vi "RealTime.vi"() -> ()   [LabVIEW 2019]
uses:
  ByteGSAPIBase/LimsTestStep/acquisitions.ctl
  <vilib>/Bytelabs/ByteChannelsSetting/ChannelSettingsLib/ChannelsRepos/ChannelsRepoXML/ChannelsRepoXML.lvclass
  C:/Program Files (x86)/National Instruments/LabVIEW 2019/vi.lib/Bytelabs/ByteChannelsSetting/ChannelSettingsLib/ChannelsRepos/ChannelsRepoBase/ChannelsRepoBase.lvclass
  TypeDef/ChannelInfo.ctl
  ByteGSAPIBase/ByteGSAPIBase.lvclass
  TypeDef/TCPMessage.ctl
  <vilib>/Bytelabs/ByteChannelsSetting/ChannelSettingsLib/ChannelsClasses/ChannelBase/ChannelBase.lvclass/ChannelBase.ctl
  <vilib>/Bytelabs/ByteChannelsSetting/ChannelSettingsLib/ChannelsClasses/ChannelAnalog/AnalogRio/AnalogRio.lvclass
  C:/Program Files (x86)/National Instruments/LabVIEW 2019/vi.lib/Bytelabs/ByteChannelsSetting/ChannelSettingsLib/ChannelsClasses/ChannelAnalog/AnalogIn/AnalogIn.lvclass
  ByteGSAPIBase/UpdateChannelsList/fields.ctl
  ByteGSAPIBase/TypeDef/StepAcquisition.ctl
  ByteGSAPIBase/TypeDef/Asset.ctl
  <vilib>/Bytelabs/ByteTCP/TCP_Class/TCP.lvclass
  <vilib>/Bytelabs/ByteSimpleQ/ByteSimpleQ/ByteSimpleQ.lvlib
  <vilib>/Bytelabs/ByteChannelsSetting/ChannelSettingsLib/ChannelsRepos/ChannelsRepoBase/ChannelsRepoBase.lvclass
  <vilib>/Bytelabs/ByteChannelsSetting/ChannelSettingsLib/ChannelsClasses/ChannelBase/ChannelBase.lvclass
panel:
  out "error out":errorcluster
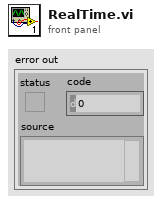
[diagram p1: front panel]
types:
  T1 = typedef "ChannelInfo.ctl" = cluster{"Tag":string, "HW Resource":string, "Raw":dbl}
  T2 = typedef "ByteGSWebAPI.lvlib/ByteGSAPIBase.lvclass/acquisitions.ctl" = cluster{"tags":cluster{"step_id":i32, "test_slug":string, "asset_slug":string}, "acquisitions":cluster{"timestamp":string, "fields":cluster{"name":string, "value":dbl}[]}[]}
  T3 = cluster{"queue out":refnum<queue>, "Acquisitions":T2, "Info":T1[], "TCP_Class":refnum<class "TCP.lvclass">, "Continous?":bool, "Duration":dbl, "ByteGSAPIBase in":refnum<class "ByteGSAPIBase.lvclass">}
  T4 = cluster{"Acquisitions":T2, "Info":T1[], "ByteGSAPIBase in":refnum<class "ByteGSAPIBase.lvclass">, "TCP_Class":refnum<class "TCP.lvclass">}
  T5 = cluster{"ByteGSAPIBase in":refnum<class "ByteGSAPIBase.lvclass">, "TCP_Class":refnum<class "TCP.lvclass">, "ChannelsRepoBase out":refnum<class "ChannelsRepoXML.lvclass">, "queue out":refnum<queue>, "Slug":string, "queue out":refnum<queue>}
  T6 = cluster{"ChannelsRepoBase out":refnum<class "ChannelsRepoXML.lvclass">, "channels":string[], "Duration":dbl, "id":i32, "prova.slug":string, "Continous?":bool, "ByteGSAPIBase in":refnum<class "ByteGSAPIBase.lvclass">}
  T7 = cluster{"timestamp":string, "fields":cluster{"name":string, "value":dbl}[]}
  T8 = typedef "TCPMessage.ctl" = cluster{"Message":string, "Data":variant}
  T9 = cluster{"timestamp":string, "fields":cluster{"name":string, "value":dbl}[]}[]
  T10 = cluster{"ChannelsRepoBase out":refnum<class "ChannelsRepoXML.lvclass">, "channels":string[], "asset_slug":string, "ByteGSAPIBase in":refnum<class "ByteGSAPIBase.lvclass">}
  T11 = typedef "ByteGSWebAPI.lvlib/ByteGSAPIBase.lvclass/fields.ctl" = cluster{"asset_slug":string, "fields":string[]}
  T12 = typedef "ByteGSWebAPI.lvlib/ByteGSAPIBase.lvclass/StepAcquisition.ctl" = cluster{"id":i32, "descrizione":string, "prova":cluster{"slug":string}, "assets":T13[], "criterio_accettazione":string, "valore_criterio_accettazione_max":dbl, "valore_criterio_accettazione_min":dbl, "udm_criterio_accettazione":string, "duration_prova":string, "udm_duration_prova":string, "valore_prova":dbl, "ordine":i32, "user":i32, "link_automation":string, "instruction_automation":string, "data_completamento_checklist":timestamp, "outcome":bool, "step_type":string, "channels":string[]}
  T13 = typedef "ByteGSWebAPI.lvlib/ByteGSAPIBase.lvclass/Asset.ctl" = cluster{"descrizione":string, "slug":string, "id":i32}
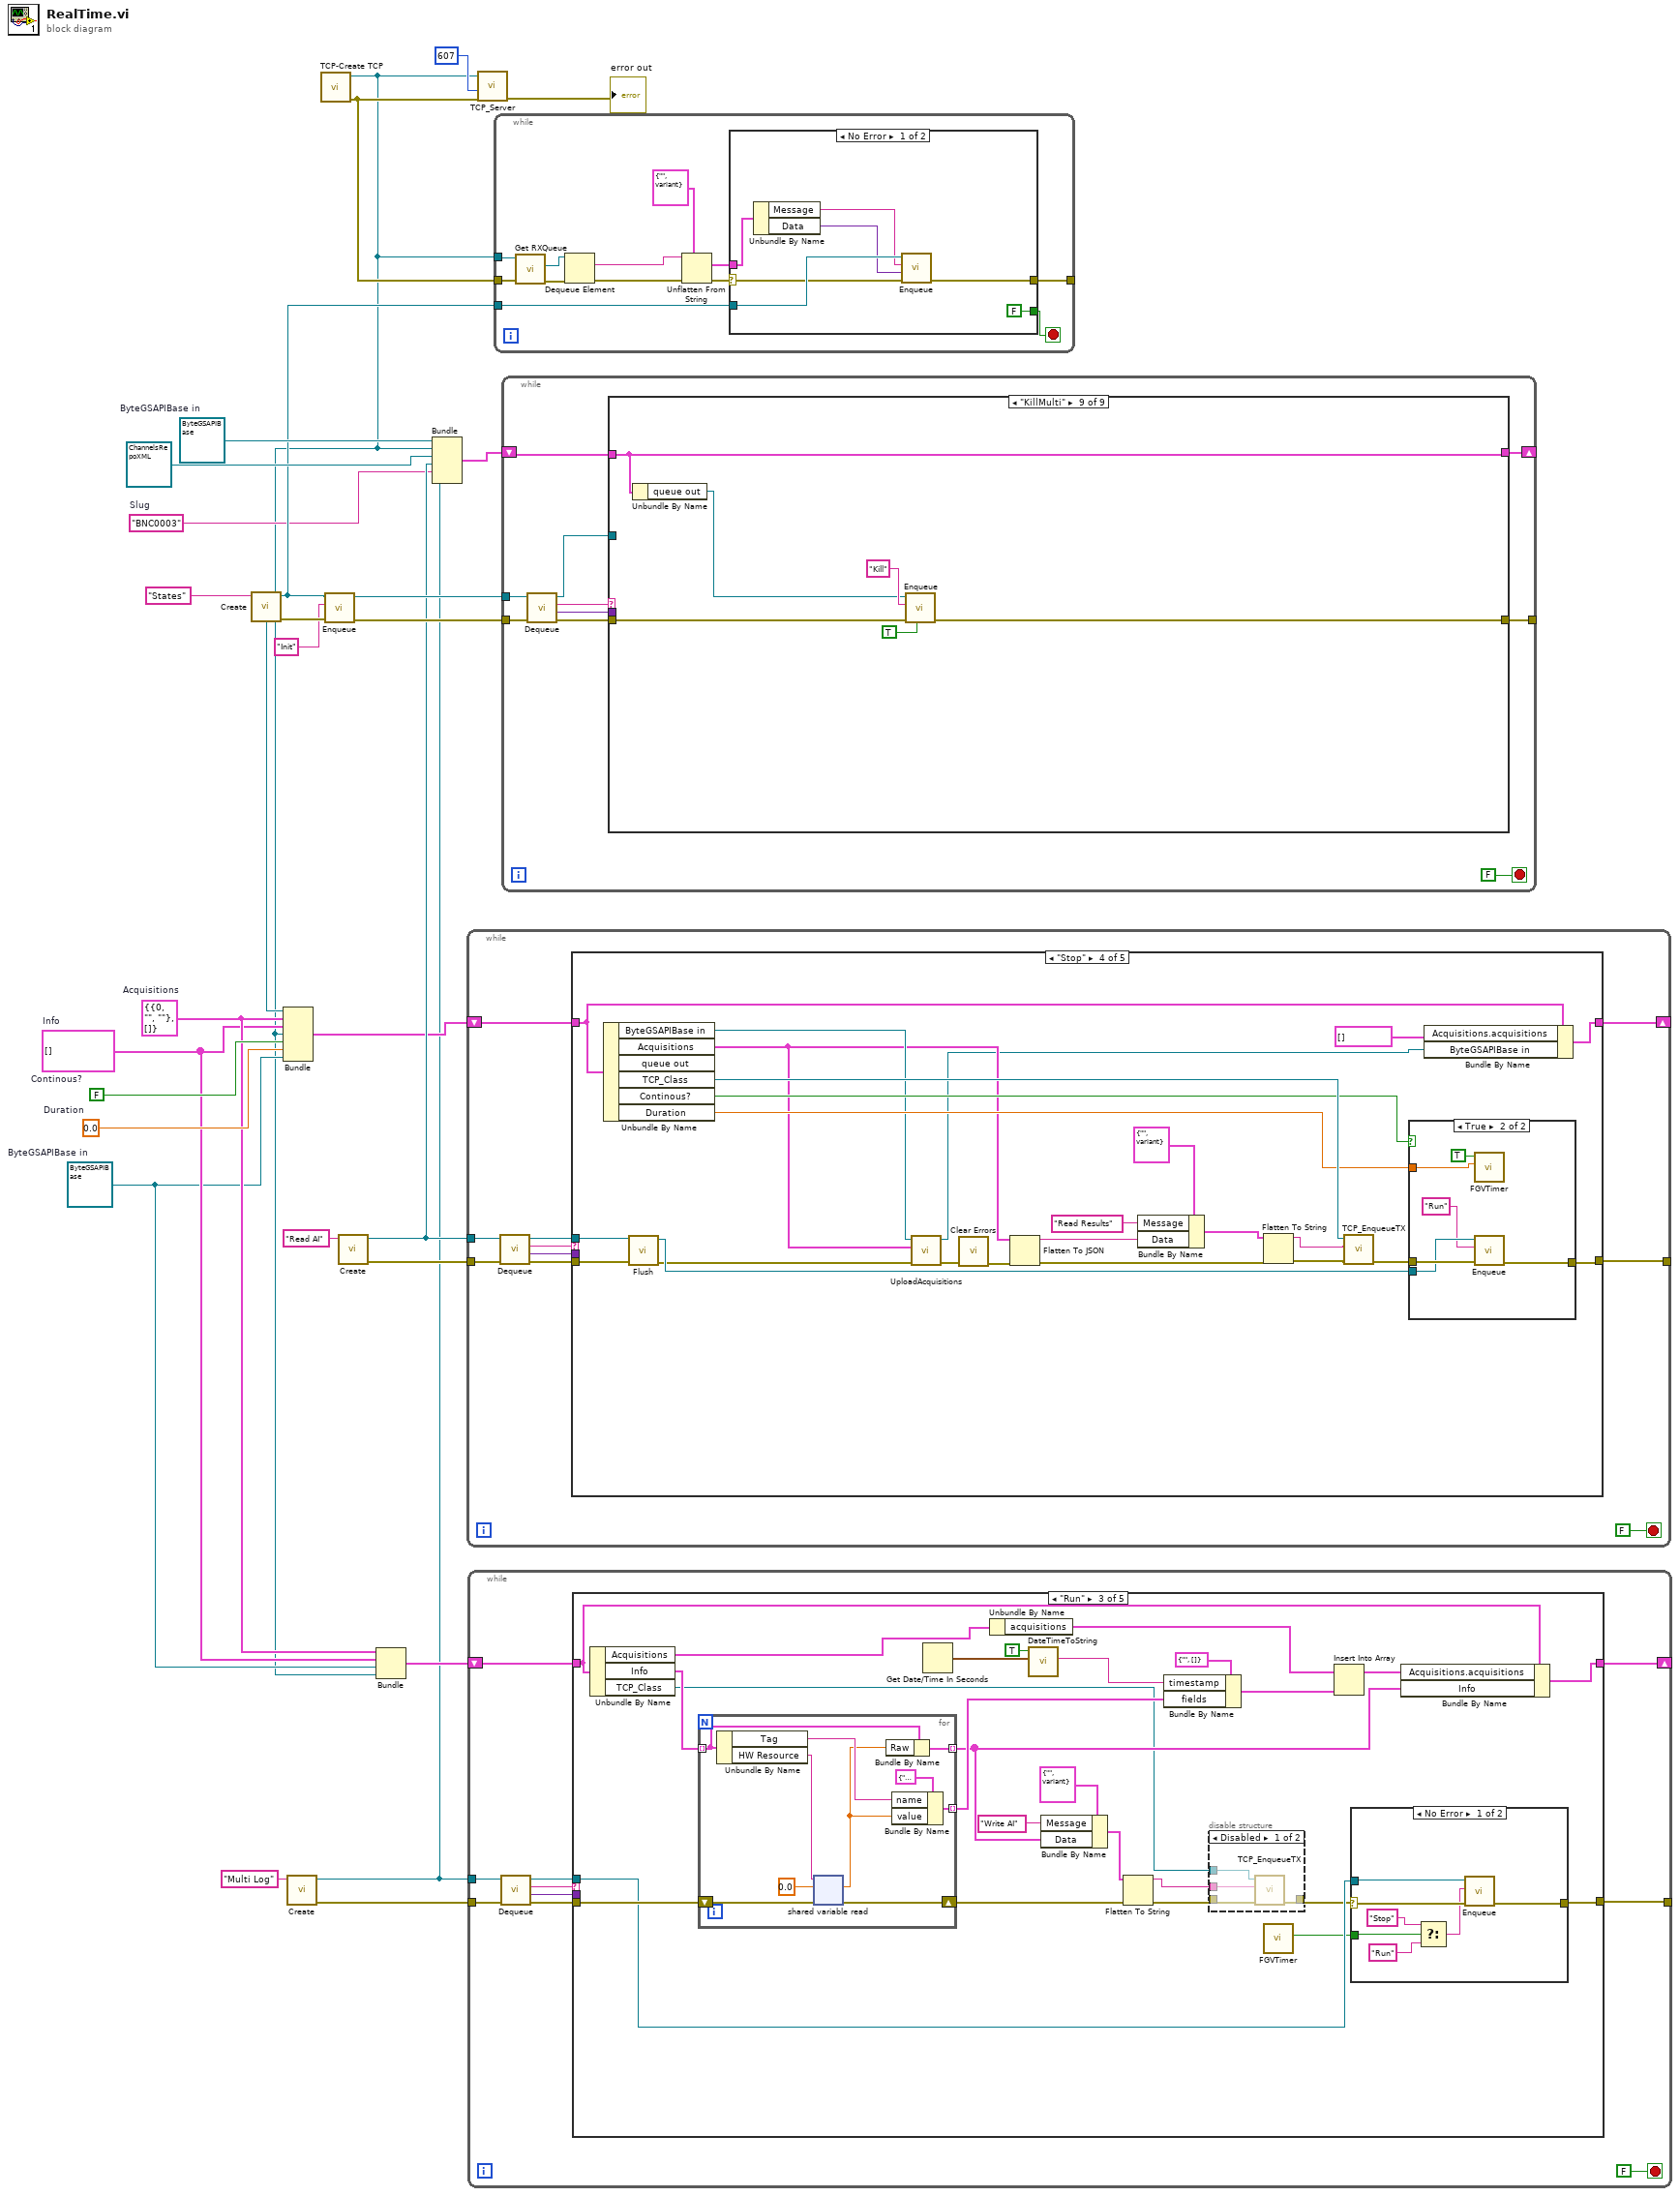
[diagram p0: block diagram]
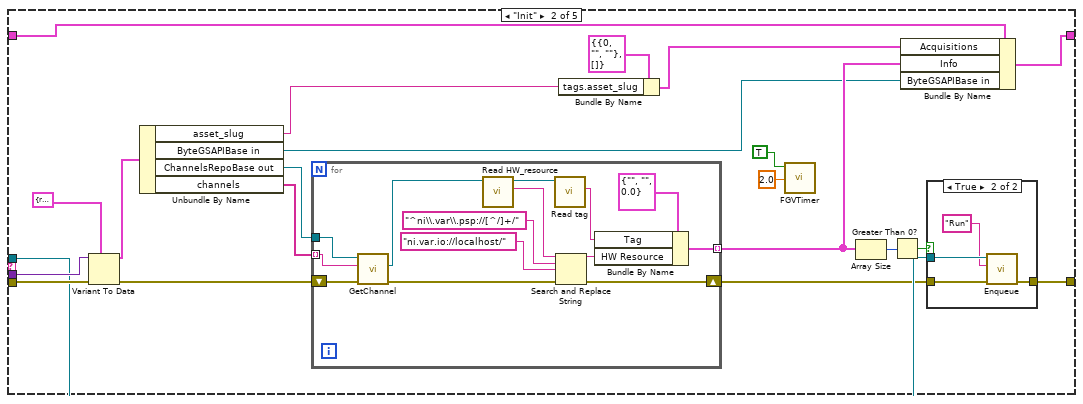
[diagram p3: hidden frame]
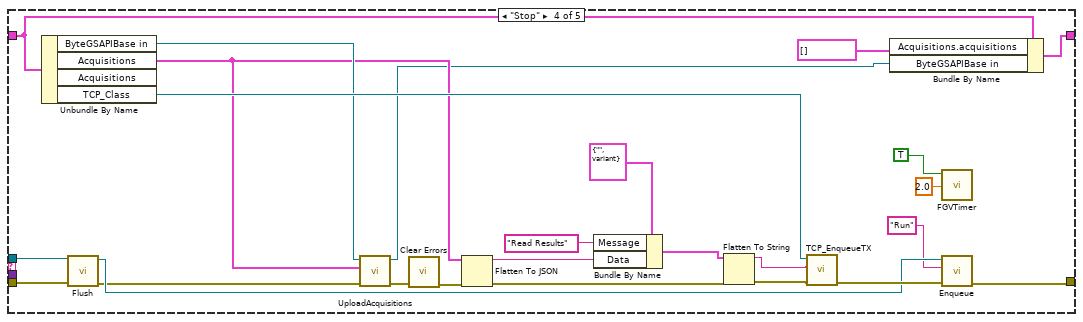
[diagram p7: hidden frame]
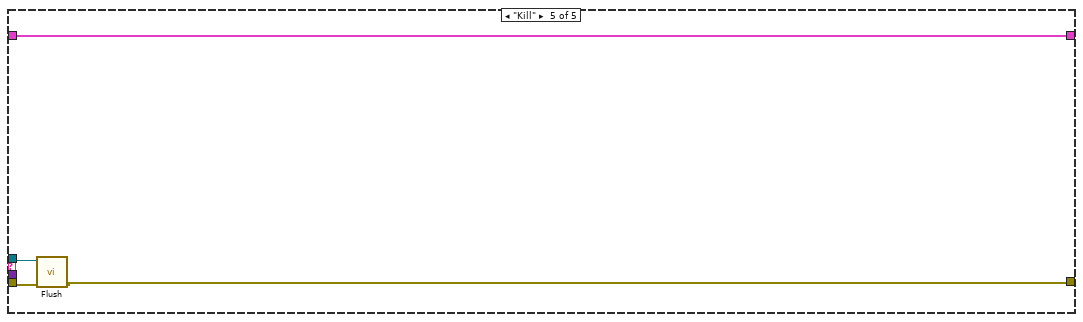
[diagram p8: hidden frame]
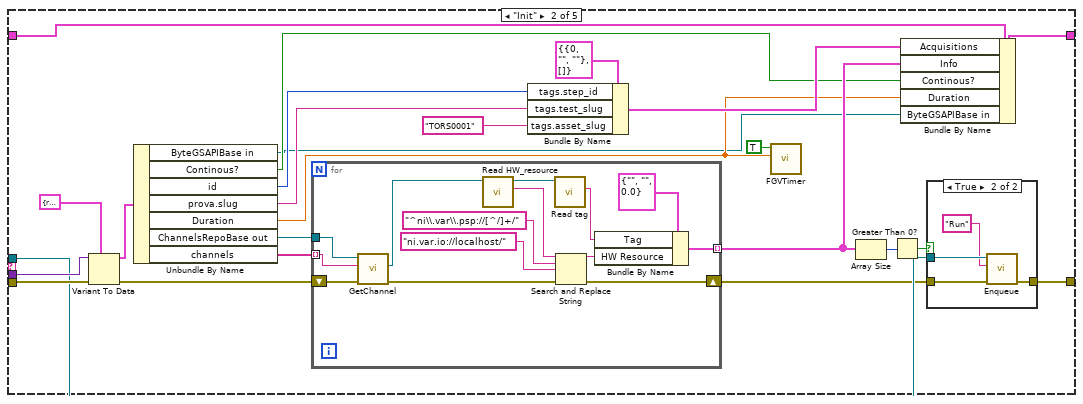
[diagram p10: hidden frame]
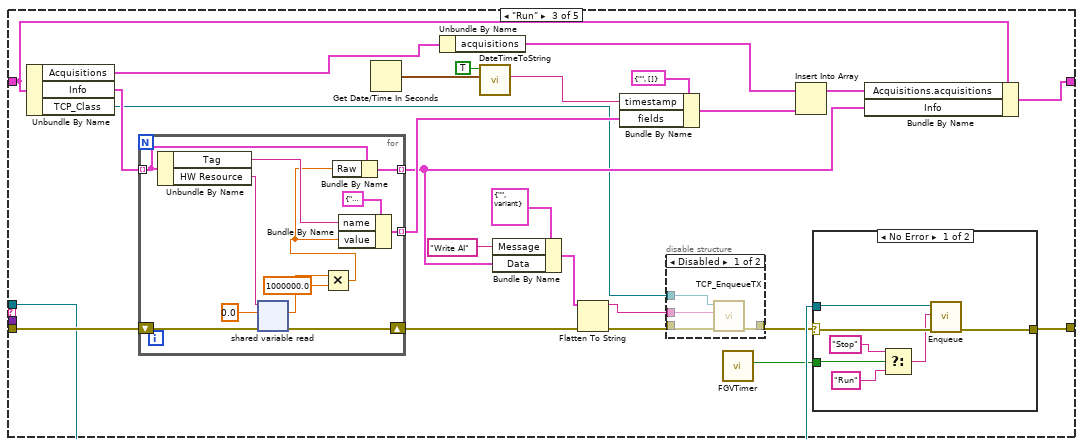
[diagram p12: hidden frame]
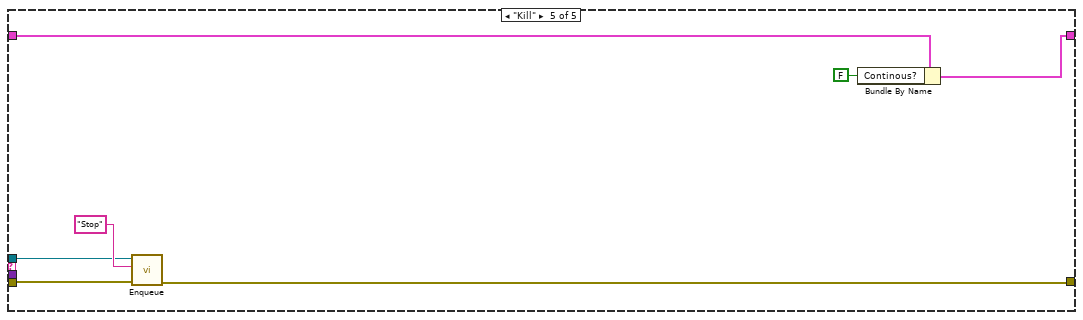
[diagram p16: hidden frame]
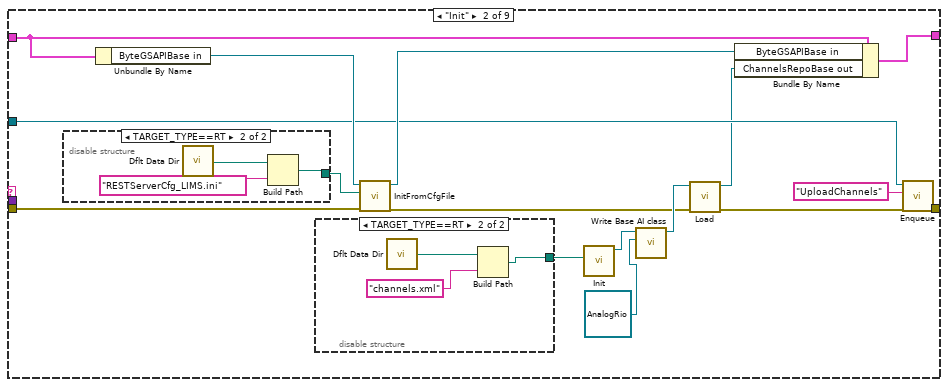
[diagram p18: hidden frame]
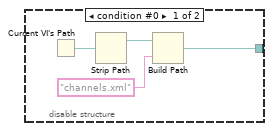
[diagram p19: hidden frame]
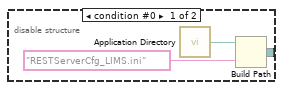
[diagram p20: hidden frame]
diagram:
  w9 = "BNC0003"  # Slug
  w4 = refnum<class "ByteGSAPIBase.lvclass"> refnum  # ByteGSAPIBase in
  w10 = 0.0  # Duration
  w11 = FALSE  # Continous?
  w5 = T1[] []  # Info
  w6 = T2 {"tags"={"step_id"=0, "test_slug"="", "asset_slug"=""}, "acquisitions"=[]}  # Acquisitions
  w17 = refnum<class "ByteGSAPIBase.lvclass"> refnum  # ByteGSAPIBase in
  n1 = call <vilib>:"Create.vi"("name (unnamed)"="States") -> ("error out"=w21:errorcluster, "queue out"=w13:refnum<queue>)  [unwired: 8 in, 1 out]
  n2 = call <vilib>:"Create.vi"("name (unnamed)"="Multi Log") -> ("error out"=w7:errorcluster, "queue out"=w1:refnum<queue>)  [unwired: 8 in, 1 out]
  n3 = call <vilib>:"TCP-Create TCP.vi"() -> ("error out"=w27:errorcluster, "TCP_Class"=w3:refnum<class "TCP.lvclass">)  [unwired: 9 in, 1 out]
  n4 = Bundle("queue out"=w13, "Acquisitions"=w6, "Info"=w5, "TCP_Class"=w3, "Continous?"=w11, "Duration"=w10, "ByteGSAPIBase in"=w4) -> (w12:T3)  [unwired: 1 in]
  n5 = call <vilib>:"Enqueue.vi"("error in (no error)"=w21, "message"="Init", "queue in"=w13) -> ("error out"=w20:errorcluster, "queue out"=w19:refnum<queue>)  [unwired: 6 in, 1 out]
  n6 = call <vilib>:"Create.vi"("name (unnamed)"="Read AI") -> ("error out"=w23:errorcluster, "queue out"=w15:refnum<queue>)  [unwired: 8 in, 1 out]
  n7 = Bundle("Acquisitions"=w6, "Info"=w5, "ByteGSAPIBase in"=w4, "TCP_Class"=w3) -> (w2:T4)  [unwired: 1 in]
  n8 = Bundle("ByteGSAPIBase in"=w17, "TCP_Class"=w3, "ChannelsRepoBase out"=refnum<class "ChannelsRepoXML.lvclass"> refnum, "queue out"=w15, "Slug"=w9, "queue out"=w1) -> (w14:T5)  [unwired: 1 in]
  n9 = while {
    tunnel: w15 -> [w37]
    shift-right: [w28] -> _
    shift-left: w12 -> [w29]
    tunnel: w23 -> [w36]
    tunnel: [w31] -> _
    stop <- FALSE stop-if-true
    n10 = call <vilib>:"Dequeue.vi"("error in (no error)"=w36, "queue in"=w37) -> ("error out"=w35:errorcluster, "data"=w33:variant, "message"=w34:string, "queue out"=w32:refnum<queue>)  [unwired: 5 in, 1 out]
    n11 = case shown="\"Stop\"" w34 {
      tunnel: w35 -> [w39 w63 w107 w155 w168]
      tunnel: w33 -> [_ w62 _ _ _]
      tunnel: w32 -> [_ w58 w106 w154 w167]
      tunnel: [w39 w57 w105 w143 w166] -> w31
      tunnel: w29 -> [w38 w48 w86 w140 w165]
      tunnel: [w38 w46 w84 w139 w163] -> w28
      frame Default {
      }
      frame "Init" {
        n12 = Variant To Data(error in=w63, type=T6 {"ChannelsRepoBase out"=refnum, "channels"=[], "Duration"=0.0, "id"=0, "prova.slug"="", "Continous?"=FALSE, "ByteGSAPIBase in"=refnum} ("output cluster"), Variant=w62) -> (data=w56:T6, error out=w61:errorcluster)
        n13 = Unbundle By Name(w56) -> ("ByteGSAPIBase in"=w40:refnum<class "ByteGSAPIBase.lvclass">, "Continous?"=w44:bool, "id"=w50:i32, "prova.slug"=w49:string, "Duration"=w42:dbl, "ChannelsRepoBase out"=w54:refnum<class "ChannelsRepoXML.lvclass">, "channels"=w55:string[])
        n14 = for {
          shift-right: [w77] -> w53
          shift-left: w61 -> [w72]
          tunnel: [w74] -> w45 mode=indexing
          tunnel: w55 -> [w70] mode=indexing
          tunnel: w54 -> [w73]
          n15 = call <vilib>:"GetChannel.vi"("error in (no error)"=w72, "tag"=w70, "ChannelsRepoBase in"=w73) -> ("error out"=w71:errorcluster, "channel"=w69:refnum<class "ChannelBase.lvclass">)  [unwired: 5 in, 2 out]
          n16 = call <vilib>:"Read HW_resource.vi"("ChannelBase in"=w69) -> ("HW_resource"=w82:string, "ChannelBase out"=w79:refnum<class "ChannelBase.lvclass">)  [unwired: 9 in]
          n17 = call <vilib>:"Read tag.vi"("ChannelBase in"=w79) -> ("tag"=w78:string)  [unwired: 9 in, 1 out]
          n18 = Search and Replace String(input string=w82, search string="^ni\\.var\\.psp://[^/]+/", replace string="ni.var.io://localhost/" ("replace string (\"\")"), error in=w71) -> (result string=w76:string, error out=w77:errorcluster)  [unwired: 4 in, 2 out]
          n19 = Bundle By Name(cluster=T1 {"Tag"="", "HW Resource"="", "Raw"=0.0} ("output cluster"), "Tag"=w78, "HW Resource"=w76) -> (w74:T1)
        }
        n20 = Bundle By Name(cluster=T2 {"tags"={"step_id"=0, "test_slug"="", "asset_slug"=""}, "acquisitions"=[]} ("Cluster"), "tags.step_id"=w50, "tags.test_slug"=w49, "tags.asset_slug"="TORS0001") -> (w47:T2)
        n21 = call "FGVTimer.vi"("set timer"=w42, "Reset"=TRUE) -> ()  [unwired: 8 in, 2 out]
        n22 = Array Size(array=w45) -> (size(s)=w60:i32)
        n23 = Greater Than 0?(x=w60) -> (x > 0?=w59:bool)
        n24 = Bundle By Name(cluster=w48, "Acquisitions"=w47, "Info"=w45, "Continous?"=w44, "Duration"=w42, "ByteGSAPIBase in"=w40) -> (w46:T3)
        n25 = case shown="True" w59 {
          tunnel: w58 -> [_ w68]
          tunnel: [w64 w66] -> w57
          tunnel: w53 -> [w64 w65]
          frame False {
          }
          frame True {
            n26 = call <vilib>:"Enqueue.vi"("error in (no error)"=w65, "message"="Run", "queue in"=w68) -> ("error out"=w66:errorcluster)  [unwired: 6 in, 2 out]
          }
        }
      }
      frame "Run" {
        n27 = Unbundle By Name(w86) -> ("Acquisitions"=w87:T2, "Info"=w88:T1[], "TCP_Class"=w83:refnum<class "TCP.lvclass">)
        n28 = for {
          shift-right: [w127] -> w94
          shift-left: w107 -> [w131]
          tunnel: w88 -> [w128] mode=indexing
          tunnel: [w126] -> w85 mode=indexing
          tunnel: [w123] -> w100 mode=indexing
          n29 = Unbundle By Name(w128) -> ("Tag"=w124:string, "HW Resource"=w129:string)
          n30 = shared-variable-read(w129, w131, 0.0) -> (w127:errorcluster, w122:dbl)  [unwired: 2 out]
          n31 = Multiply(x=w122, y=1000000.0) -> (x*y=w120:dbl)
          n32 = Bundle By Name(cluster=w128, "Raw"=w120) -> (w126:T1)
          n33 = Bundle By Name(cluster=cluster{"name":string, "value":dbl} {"name"="", "value"=0.0} ("fields"), "name"=w124, "value"=w120) -> (w123:cluster{"name":string, "value":dbl})
        }
        n34 = Get Date/Time In Seconds() -> (seconds since 1Jan1904=w91:timestamp)
        n35 = Unbundle By Name(w87) -> ("acquisitions"=w98:T9)
        n36 = call "DateTimeToString.vi"("current time"=w91, "include Time?"=TRUE) -> ("date string"=w90:string)  [unwired: 8 in, 1 out]
        n37 = Bundle By Name(cluster=T8 {"Message"="", "Data"=variant}, "Message"="Write AI", "Data"=w85) -> (w103:T8)
        n38 = Flatten To String(anything=w103, error in (no error)=w94) -> (data string=w95:string, error out=w96:errorcluster)  [unwired: 2 in, 1 out]
        n39 = Bundle By Name(cluster=T7 {"timestamp"="", "fields"=[]} ("acquisition"), "timestamp"=w90, "fields"=w100) -> (w99:T7)
        n40 = disable-structure shown="Disabled" {
          disable-tunnel: w96 -> [w111 _]
          disable-tunnel: w95 -> [w110 _]
          disable-tunnel: [w109 _] -> w92
          disable-tunnel: w83 -> [w108 _]
          frame Disabled {
            n41 = call-dynamic "TCP_EnqueueTX.vi"("error in (no error)"=w111, "Msg to Transmit"=w110, "TCP in"=w108) -> ("error out"=w109:errorcluster)  [unwired: 7 in, 1 out]
          }
          frame Enabled {
          }
        }
        n42 = call "FGVTimer.vi"() -> ("Elapsed?"=w93:bool)  [unwired: 10 in, 1 out]
        n43 = Insert Into Array(array=w98, new element=w99) -> (w97:T9)  [unwired: 1 in]
        n44 = case shown="No Error" w92 {
          selector: w92 -> [w118 w119]
          tunnel: w106 -> [w116 _]
          tunnel: [w117 w119] -> w105
          tunnel: w93 -> [w115 _]
          frame No Error {
            n45 = Select(t="Stop" ("message"), s=w115, f="Run" ("message")) -> (s? t:f=w112:string)
            n46 = call <vilib>:"Enqueue.vi"("error in (no error)"=w118, "message"=w112, "queue in"=w116) -> ("error out"=w117:errorcluster)  [unwired: 6 in, 2 out]
          }
          frame Error {
          }
        }
        n47 = Bundle By Name(cluster=w86, "Acquisitions.acquisitions"=w97, "Info"=w85) -> (w84:T3)
      }
      frame "Stop" {
        n48 = Unbundle By Name(w140) -> ("ByteGSAPIBase in"=w136:refnum<class "ByteGSAPIBase.lvclass">, "Acquisitions"=w135:T2, "TCP_Class"=w146:refnum<class "TCP.lvclass">, "Continous?"=w145:bool, "Duration"=w141:dbl)  [unwired: 1 out]
        n49 = call <vilib>:"Flush.vi"("error in"=w155, "queue in"=w154) -> ("error out"=w137:errorcluster, "queue out"=w142:refnum<queue>)  [unwired: 8 in]
        n50 = call-dynamic "UploadAcquisitions.vi"("error in (no error)"=w137, "Acquisitions"=w135, "ByteGSAPIBase in"=w136) -> ("error out"=w133:errorcluster, "ByteGSAPIBase out"=w134:refnum<class "ByteGSAPIBase.lvclass">)  [unwired: 7 in]
        n51 = call <vilib>:"Clear Errors.vi"("error in (no error)"=w133) -> ("error out"=w132:errorcluster)  [unwired: 5 in, 1 out]
        n52 = Flatten To JSON(anything=w135, error in (no error)=w132) -> (JSON string=w147:string, 11:w148:errorcluster)  [unwired: 1 in]
        n53 = Bundle By Name(cluster=T8 {"Message"="", "Data"=variant}, "Message"="Read Results", "Data"=w147) -> (w152:T8)
        n54 = Flatten To String(anything=w152, error in (no error)=w148) -> (data string=w149:string, error out=w150:errorcluster)  [unwired: 2 in, 1 out]
        n55 = call-dynamic "TCP_EnqueueTX.vi"("error in (no error)"=w150, "Msg to Transmit"=w149, "TCP in"=w146) -> ("error out"=w144:errorcluster)  [unwired: 7 in, 1 out]
        n56 = case shown="True" w145 {
          tunnel: w144 -> [w156 w162]
          tunnel: [w156 w161] -> w143
          tunnel: w142 -> [_ w160]
          tunnel: w141 -> [_ w157]
          frame False {
          }
          frame True {
            n57 = call "FGVTimer.vi"("set timer"=w157, "Reset"=TRUE) -> ()  [unwired: 8 in, 2 out]
            n58 = call <vilib>:"Enqueue.vi"("error in (no error)"=w162, "message"="Run", "queue in"=w160) -> ("error out"=w161:errorcluster)  [unwired: 6 in, 2 out]
          }
        }
        n59 = Bundle By Name(cluster=w140, "Acquisitions.acquisitions"=T9 [], "ByteGSAPIBase in"=w134) -> (w139:T3)
      }
      frame "Kill" {
        n60 = call <vilib>:"Enqueue.vi"("error in (no error)"=w168, "message"="Stop", "queue in"=w167) -> ("error out"=w166:errorcluster)  [unwired: 6 in, 2 out]
        n61 = Bundle By Name(cluster=w165, "Continous?"=FALSE) -> (w163:T3)
      }
    }
  }
  n62 = while {
    tunnel: w1 -> [w179]
    shift-right: [w170] -> _
    shift-left: w2 -> [w171]
    tunnel: w7 -> [w178]
    tunnel: [w173] -> _
    stop <- FALSE stop-if-true
    n63 = call <vilib>:"Dequeue.vi"("error in (no error)"=w178, "queue in"=w179) -> ("error out"=w177:errorcluster, "data"=w175:variant, "message"=w176:string, "queue out"=w174:refnum<queue>)  [unwired: 5 in, 1 out]
    n64 = case shown="\"Run\"" w176 {
      tunnel: w177 -> [w181 w202 w246 w293 w296]
      tunnel: w175 -> [_ w201 _ _ _]
      tunnel: w174 -> [_ w197 w245 w292 w295]
      tunnel: [w181 w196 w244 w282 w294] -> w173
      tunnel: w171 -> [w180 w190 w225 w280 w297]
      tunnel: [w180 w189 w223 w279 w297] -> w170
      frame Default {
      }
      frame "Init" {
        n65 = Variant To Data(error in=w202, type=T10 {"ChannelsRepoBase out"=refnum, "channels"=[], "asset_slug"="", "ByteGSAPIBase in"=refnum} ("output cluster"), Variant=w201) -> (data=w195:T10, error out=w200:errorcluster)
        n66 = Unbundle By Name(w195) -> ("asset_slug"=w184:string, "ByteGSAPIBase in"=w187:refnum<class "ByteGSAPIBase.lvclass">, "ChannelsRepoBase out"=w193:refnum<class "ChannelsRepoXML.lvclass">, "channels"=w194:string[])
        n67 = for {
          shift-right: [w216] -> w192
          shift-left: w200 -> [w211]
          tunnel: [w213] -> w188 mode=indexing
          tunnel: w194 -> [w209] mode=indexing
          tunnel: w193 -> [w212]
          n68 = call <vilib>:"GetChannel.vi"("error in (no error)"=w211, "tag"=w209, "ChannelsRepoBase in"=w212) -> ("error out"=w210:errorcluster, "channel"=w208:refnum<class "ChannelBase.lvclass">)  [unwired: 5 in, 2 out]
          n69 = call <vilib>:"Read HW_resource.vi"("ChannelBase in"=w208) -> ("HW_resource"=w221:string, "ChannelBase out"=w218:refnum<class "ChannelBase.lvclass">)  [unwired: 9 in]
          n70 = call <vilib>:"Read tag.vi"("ChannelBase in"=w218) -> ("tag"=w217:string)  [unwired: 9 in, 1 out]
          n71 = Search and Replace String(input string=w221, search string="^ni\\.var\\.psp://[^/]+/", replace string="ni.var.io://localhost/" ("replace string (\"\")"), error in=w210) -> (result string=w215:string, error out=w216:errorcluster)  [unwired: 4 in, 2 out]
          n72 = Bundle By Name(cluster=T1 {"Tag"="", "HW Resource"="", "Raw"=0.0} ("output cluster"), "Tag"=w217, "HW Resource"=w215) -> (w213:T1)
        }
        n73 = Bundle By Name(cluster=T2 {"tags"={"step_id"=0, "test_slug"="", "asset_slug"=""}, "acquisitions"=[]} ("Cluster"), "tags.asset_slug"=w184) -> (w183:T2)
        n74 = call "FGVTimer.vi"("set timer"=2.0, "Reset"=TRUE) -> ()  [unwired: 8 in, 2 out]
        n75 = Array Size(array=w188) -> (size(s)=w199:i32)
        n76 = Greater Than 0?(x=w199) -> (x > 0?=w198:bool)
        n77 = Bundle By Name(cluster=w190, "Acquisitions"=w183, "Info"=w188, "ByteGSAPIBase in"=w187) -> (w189:T4)
        n78 = case shown="True" w198 {
          tunnel: w197 -> [_ w207]
          tunnel: [w203 w205] -> w196
          tunnel: w192 -> [w203 w204]
          frame False {
          }
          frame True {
            n79 = call <vilib>:"Enqueue.vi"("error in (no error)"=w204, "message"="Run", "queue in"=w207) -> ("error out"=w205:errorcluster)  [unwired: 6 in, 2 out]
          }
        }
      }
      frame "Run" {
        n80 = Unbundle By Name(w225) -> ("Acquisitions"=w226:T2, "Info"=w227:T1[], "TCP_Class"=w222:refnum<class "TCP.lvclass">)
        n81 = for {
          shift-right: [w264] -> w233
          shift-left: w246 -> [w268]
          tunnel: w227 -> [w265] mode=indexing
          tunnel: [w263] -> w224 mode=indexing
          tunnel: [w260] -> w239 mode=indexing
          n82 = Unbundle By Name(w265) -> ("Tag"=w261:string, "HW Resource"=w266:string)
          n83 = shared-variable-read(w266, w268, 0.0) -> (w264:errorcluster, w259:dbl)  [unwired: 2 out]
          n84 = Bundle By Name(cluster=w265, "Raw"=w259) -> (w263:T1)
          n85 = Bundle By Name(cluster=cluster{"name":string, "value":dbl} {"name"="", "value"=0.0} ("fields"), "name"=w261, "value"=w259) -> (w260:cluster{"name":string, "value":dbl})
        }
        n86 = Get Date/Time In Seconds() -> (seconds since 1Jan1904=w230:timestamp)
        n87 = Unbundle By Name(w226) -> ("acquisitions"=w237:T9)
        n88 = call "DateTimeToString.vi"("current time"=w230, "include Time?"=TRUE) -> ("date string"=w229:string)  [unwired: 8 in, 1 out]
        n89 = Bundle By Name(cluster=T8 {"Message"="", "Data"=variant}, "Message"="Write AI", "Data"=w224) -> (w242:T8)
        n90 = Flatten To String(anything=w242, error in (no error)=w233) -> (data string=w234:string, error out=w235:errorcluster)  [unwired: 2 in, 1 out]
        n91 = Bundle By Name(cluster=T7 {"timestamp"="", "fields"=[]} ("acquisition"), "timestamp"=w229, "fields"=w239) -> (w238:T7)
        n92 = disable-structure shown="Disabled" {
          disable-tunnel: w235 -> [w250 _]
          disable-tunnel: w234 -> [w249 _]
          disable-tunnel: [w248 _] -> w231
          disable-tunnel: w222 -> [w247 _]
          frame Disabled {
            n93 = call-dynamic "TCP_EnqueueTX.vi"("error in (no error)"=w250, "Msg to Transmit"=w249, "TCP in"=w247) -> ("error out"=w248:errorcluster)  [unwired: 7 in, 1 out]
          }
          frame Enabled {
          }
        }
        n94 = call "FGVTimer.vi"() -> ("Elapsed?"=w232:bool)  [unwired: 10 in, 1 out]
        n95 = Insert Into Array(array=w237, new element=w238) -> (w236:T9)  [unwired: 1 in]
        n96 = case shown="No Error" w231 {
          selector: w231 -> [w257 w258]
          tunnel: w245 -> [w255 _]
          tunnel: [w256 w258] -> w244
          tunnel: w232 -> [w254 _]
          frame No Error {
            n97 = Select(t="Stop" ("message"), s=w254, f="Run" ("message")) -> (s? t:f=w251:string)
            n98 = call <vilib>:"Enqueue.vi"("error in (no error)"=w257, "message"=w251, "queue in"=w255) -> ("error out"=w256:errorcluster)  [unwired: 6 in, 2 out]
          }
          frame Error {
          }
        }
        n99 = Bundle By Name(cluster=w225, "Acquisitions.acquisitions"=w236, "Info"=w224) -> (w223:T4)
      }
      frame "Stop" {
        n100 = Unbundle By Name(w280) -> ("ByteGSAPIBase in"=w276:refnum<class "ByteGSAPIBase.lvclass">, "Acquisitions"=w275:T2, "TCP_Class"=w284:refnum<class "TCP.lvclass">)  [unwired: 1 out]
        n101 = call <vilib>:"Flush.vi"("error in"=w293, "queue in"=w292) -> ("error out"=w277:errorcluster, "queue out"=w281:refnum<queue>)  [unwired: 8 in]
        n102 = call-dynamic "UploadAcquisitions.vi"("error in (no error)"=w277, "Acquisitions"=w275, "ByteGSAPIBase in"=w276) -> ("error out"=w273:errorcluster, "ByteGSAPIBase out"=w274:refnum<class "ByteGSAPIBase.lvclass">)  [unwired: 7 in]
        n103 = call <vilib>:"Clear Errors.vi"("error in (no error)"=w273) -> ("error out"=w272:errorcluster)  [unwired: 5 in, 1 out]
        n104 = Flatten To JSON(anything=w275, error in (no error)=w272) -> (JSON string=w285:string, 11:w286:errorcluster)  [unwired: 1 in]
        n105 = Bundle By Name(cluster=T8 {"Message"="", "Data"=variant}, "Message"="Read Results", "Data"=w285) -> (w290:T8)
        n106 = Flatten To String(anything=w290, error in (no error)=w286) -> (data string=w287:string, error out=w288:errorcluster)  [unwired: 2 in, 1 out]
        n107 = call-dynamic "TCP_EnqueueTX.vi"("error in (no error)"=w288, "Msg to Transmit"=w287, "TCP in"=w284) -> ("error out"=w283:errorcluster)  [unwired: 7 in, 1 out]
        n108 = Bundle By Name(cluster=w280, "Acquisitions.acquisitions"=T9 [], "ByteGSAPIBase in"=w274) -> (w279:T4)
        n109 = call "FGVTimer.vi"("set timer"=2.0, "Reset"=TRUE) -> ()  [unwired: 8 in, 2 out]
        n110 = call <vilib>:"Enqueue.vi"("error in (no error)"=w283, "message"="Run", "queue in"=w281) -> ("error out"=w282:errorcluster)  [unwired: 6 in, 2 out]
      }
      frame "Kill" {
        n111 = call <vilib>:"Flush.vi"("error in"=w296, "queue in"=w295) -> ("error out"=w294:errorcluster)  [unwired: 8 in, 1 out]
      }
    }
  }
  n112 = call <vilib>:"TCP_Server.vi"("error in (no error)"=w27, "TxPort"=u16 607, "TCP.lvlib:TCP.lvclass"=w3) -> ("error out"=→"error out":errorcluster)  [unwired: 8 in]
  n113 = while {
    tunnel: w3 -> [w301]
    tunnel: w13 -> [w309]
    tunnel: w27 -> [w302]
    tunnel: [w305] -> _
    stop <- w298 stop-if-true
    # "Receiver"
    n114 = call-dynamic "Get RXQueue.vi"("error in (no error)"=w302, "TCP in"=w301) -> ("error out"=w304:errorcluster, "RX"=w303:refnum<queue>)  [unwired: 7 in, 1 out]
    n115 = Dequeue Element(queue=w303, error in (no error)=w304) -> (element=w299:string, error out=w300:errorcluster)  [unwired: 1 in, 2 out]
    n116 = Unflatten From String(type=T8 {"Message"="", "Data"=variant}, binary string=w299, error in (no error)=w300) -> (value=w306:T8, error out=w308:errorcluster)  [unwired: 2 in, 1 out]
    n117 = case shown="No Error" w308 {
      selector: w308 -> [w315 _]
      tunnel: w309 -> [w316 _]
      tunnel: w306 -> [w314 _]
      tunnel: [w311 _] -> w305
      tunnel: [FALSE FALSE] -> w298
      frame No Error {
        n118 = Unbundle By Name(w314) -> ("Message"=w312:string, "Data"=w313:variant)
        n119 = call <vilib>:"Enqueue.vi"("error in (no error)"=w315, "data"=w313, "message"=w312, "queue in"=w316) -> ("error out"=w311:errorcluster)  [unwired: 5 in, 2 out]
      }
      frame Error {
      }
    }
  }
  n120 = while {
    tunnel: w19 -> [w326]
    shift-right: [w319] -> _
    shift-left: w14 -> [w320]
    tunnel: w20 -> [w327]
    tunnel: [w321] -> _
    stop <- FALSE stop-if-true
    n121 = call <vilib>:"Dequeue.vi"("error in (no error)"=w327, "queue in"=w326) -> ("error out"=w325:errorcluster, "data"=w324:variant, "message"=w323:string, "queue out"=w318:refnum<queue>)  [unwired: 5 in, 1 out]
    n122 = case shown="\"KillMulti\"" w323 {
      tunnel: w325 -> [w329 w345 w367 w385 w418 w438 w450 w470 w475]
      tunnel: w324 -> [_ _ _ _ w417 _ w449 _ _]
      tunnel: [w329 w338 w359 w386 w414 w437 w444 w457 w474] -> w321
      tunnel: w320 -> [w328 w342 w362 w394 w410 w435 w442 w468 w473]
      tunnel: [w328 w340 w360 w393 w410 w435 w441 w467 w473] -> w319
      tunnel: w318 -> [_ w339 _ w391 _ _ _ _ _]
      frame Default {
      }
      frame "Init" {
        n123 = disable-structure shown="TARGET_TYPE==RT" {
          disable-tunnel: [w353 w356] -> w344
          frame condition #0 {
            n124 = call <vilib>:"Application Directory.vi"() -> ("Application Directory"=w354:path)
            n125 = Build Path(base path=w354, name or relative path="RESTServerCfg_LIMS.ini") -> (appended path=w353:path)
          }
          frame condition #1 (active) {
            n126 = call <vilib>:"Dflt Data Dir.vi"() -> ("App:Default Data Directory"=w358:path)
            n127 = Build Path(base path=w358, name or relative path="RESTServerCfg_LIMS.ini") -> (appended path=w356:path)
          }
        }
        n128 = Unbundle By Name(w342) -> ("ByteGSAPIBase in"=w343:refnum<class "ByteGSAPIBase.lvclass">)
        n129 = disable-structure shown="TARGET_TYPE==RT" {
          disable-tunnel: [w346 w351] -> w336
          frame condition #0 {
            n130 = Current VI's Path() -> (path=w348:path)
            n131 = Strip Path(path=w348) -> (stripped path=w347:path)  [unwired: 1 out]
            n132 = Build Path(base path=w347, name or relative path="channels.xml") -> (appended path=w346:path)
          }
          frame condition #1 (active) {
            n133 = call <vilib>:"Dflt Data Dir.vi"() -> ("App:Default Data Directory"=w352:path)
            n134 = Build Path(base path=w352, name or relative path="channels.xml") -> (appended path=w351:path)
          }
        }
        n135 = call-dynamic "InitFromCfgFile.vi"("error in (no error)"=w345, "configuration file path"=w344, "ByteGSAPIBase in"=w343) -> ("error out"=w331:errorcluster, "ByteGSAPIBase out"=w341:refnum<class "ByteGSAPIBase.lvclass">)  [unwired: 7 in]
        n136 = call <vilib>:"Init.vi"("XML file path"=w336) -> ("ChannelsRepoXML out"=w333:refnum<class "ChannelsRepoXML.lvclass">)  [unwired: 10 in]
        n137 = call-dynamic "Write Base AI class.vi"("ChannelsClasses.lvlib:AnalogIn.lvclass"=refnum<class "AnalogRio.lvclass"> refnum ("ChannelSettings.lvlib:ChannelsClasses.lvlib:AnalogRio.lvclass"), "ChannelsRepoBase in"=w333) -> ("ChannelsRepoBase out"=w332:refnum<class "ChannelsRepoXML.lvclass">)  [unwired: 9 in]
        n138 = call <vilib>:"Load.vi"("error in (no error)"=w331, "ChannelsRepoBase in"=w332) -> ("error out"=w335:errorcluster, "ChannelsRepoBase out"=w334:refnum<class "ChannelsRepoXML.lvclass">)  [unwired: 7 in, 1 out]
        n139 = Bundle By Name(cluster=w342, "ByteGSAPIBase in"=w341, "ChannelsRepoBase out"=w334) -> (w340:T5)
        n140 = call <vilib>:"Enqueue.vi"("error in (no error)"=w335, "message"="UploadChannels", "queue in"=w339) -> ("error out"=w338:errorcluster)  [unwired: 6 in, 2 out]
      }
      frame "UploadChannels" {
        n141 = Unbundle By Name(w362) -> ("ByteGSAPIBase in"=w364:refnum<class "ByteGSAPIBase.lvclass">, "TCP_Class"=w363:refnum<class "TCP.lvclass">, "ChannelsRepoBase out"=w365:refnum<class "ChannelsRepoXML.lvclass">, "Slug"=w366:string)
        n142 = call <vilib>:"SortTagsByParentAndType.vi"("ChannelsRepoBase in"=w365) -> ("sorted tags"=w376:string[])  [unwired: 8 in, 2 out]
        n143 = Bundle By Name(cluster=T11 {"asset_slug"="", "fields"=[]} ("Channels"), "asset_slug"=w366, "fields"=w376) -> (w369:T11)
        n144 = disable-structure shown="Enabled" {
          disable-tunnel: w367 -> [w381 _]
          disable-tunnel: [w380 _] -> w370
          disable-tunnel: w364 -> [w379 _]
          disable-tunnel: w369 -> [w378 _]
          disable-tunnel: [w377 _] -> w361
          frame Enabled {
            n145 = call "UpdateChannelsList.vi"("error in (no error)"=w381, "Channels"=w378, "ByteGSAPIBase in"=w379) -> ("error out"=w380:errorcluster, "ByteGSAPIBase out"=w377:refnum<class "ByteGSAPIBase.lvclass">)  [unwired: 7 in]
          }
          frame Disabled {
          }
        }
        n146 = Bundle By Name(cluster=T8 {"Message"="", "Data"=variant} ("Cluster"), "Message"="update_channels_list", "Data"=w369) -> (w372:T8)
        n147 = Flatten To String(anything=w372, error in (no error)=w370) -> (data string=w371:string, error out=w373:errorcluster)  [unwired: 2 in, 1 out]
        n148 = call-dynamic "TCP_EnqueueTX.vi"("error in (no error)"=w373, "Msg to Transmit"=w371, "TCP in"=w363) -> ("error out"=w359:errorcluster)  [unwired: 7 in, 1 out]
        n149 = Bundle By Name(cluster=w362, "ByteGSAPIBase in"=w361) -> (w360:T5)
      }
      frame "Load" {
        n150 = disable-structure shown="TARGET_TYPE==RT" {
          disable-tunnel: [w395 w401] -> w389
          frame condition #0 {
            n151 = Current VI's Path() -> (path=w397:path)
            n152 = Strip Path(path=w397) -> (stripped path=w396:path)  [unwired: 1 out]
            n153 = Build Path(base path=w396, name or relative path="channels.xml") -> (appended path=w395:path)
          }
          frame condition #1 (active) {
            n154 = call <vilib>:"Dflt Data Dir.vi"() -> ("App:Default Data Directory"=w399:path)
            n155 = Build Path(base path=w399, name or relative path="channels.xml") -> (appended path=w401:path)
          }
        }
        n156 = call <vilib>:"Init.vi"("XML file path"=w389) -> ("ChannelsRepoXML out"=w384:refnum<class "ChannelsRepoXML.lvclass">)  [unwired: 10 in]
        n157 = call-dynamic "Write Base AI class.vi"("ChannelsClasses.lvlib:AnalogIn.lvclass"=refnum<class "AnalogRio.lvclass"> refnum ("ChannelSettings.lvlib:ChannelsClasses.lvlib:AnalogRio.lvclass"), "ChannelsRepoBase in"=w384) -> ("ChannelsRepoBase out"=w383:refnum<class "ChannelsRepoXML.lvclass">)  [unwired: 9 in]
        n158 = call <vilib>:"Load.vi"("error in (no error)"=w385, "ChannelsRepoBase in"=w383) -> ("error out"=w392:errorcluster, "ChannelsRepoBase out"=w387:refnum<class "ChannelsRepoXML.lvclass">)  [unwired: 7 in, 1 out]
        n159 = call <vilib>:"Enqueue.vi"("error in (no error)"=w392, "message"="UploadChannels", "queue in"=w391) -> ("error out"=w388:errorcluster)  [unwired: 6 in, 2 out]
        n160 = call <vilib>:"Clear Errors.vi"("error in (no error)"=w388) -> ("error out"=w386:errorcluster)  [unwired: 5 in, 1 out]
        n161 = Bundle By Name(cluster=w394, "ChannelsRepoBase out"=w387) -> (w393:T5)
      }
      frame "Start Step List" {
        n162 = Variant To Data(error in=w418, type=cluster{"Continous?":bool, "StepList":T12} {"Continous?"=FALSE, "StepList"={"id"=0, "descrizione"="", "prova"={"slug"=""}, "assets"=[], "criterio_accettazione"="", "valore_criterio_accettazione_max"=0.0, "valore_criterio_accettazione_min"=0.0, "udm_criterio_accettazione"="", "duration_prova"="", "udm_duration_prova"="", "valore_prova"=0.0, "ordine"=0, "user"=0, "link_automation"="", "instruction_automation"="", "data_completamento_checklist"=timestamp(0 s since 1904-01-01), "outcome"=FALSE, "step_type"="", "channels"=[]}}, Variant=w417) -> (data=w405:cluster{"Continous?":bool, "StepList":T12}, error out=w415:errorcluster)
        n163 = Unbundle By Name(w410) -> ("ByteGSAPIBase in"=w402:refnum<class "ByteGSAPIBase.lvclass">, "ChannelsRepoBase out"=w411:refnum<class "ChannelsRepoXML.lvclass">, "queue out"=w409:refnum<queue>)
        n164 = Unbundle By Name(w405) -> ("StepList"=w404:T12, "Continous?"=w403:bool)
        n165 = Unbundle By Name(w404) -> ("step_type"=w416:string, "channels"=w413:string[], "instruction_automation"=w412:string, "id"=w408:i32, "prova.slug"=w407:string)
        n166 = case shown="\"Read AI\"" w416 {
          tunnel: w415 -> [w419 w433]
          tunnel: [w419 w432] -> w414
          tunnel: w413 -> [_ w430]
          tunnel: w412 -> [_ w428]
          tunnel: w411 -> [_ w425]
          tunnel: w409 -> [_ w424]
          tunnel: w408 -> [_ w423]
          tunnel: w407 -> [_ w422]
          tunnel: w403 -> [_ w421]
          tunnel: w402 -> [_ w420]
          frame Default {
          }
          frame "Read AI" {
            n167 = Fract/Exp String To Number(string=w428) -> (number=w427:dbl)  [unwired: 3 in, 1 out]
            n168 = Bundle(cluster=T6 {"ChannelsRepoBase out"=refnum, "channels"=[], "Duration"=0.0, "id"=0, "prova.slug"="", "Continous?"=FALSE, "ByteGSAPIBase in"=refnum} ("output cluster"), "ChannelsRepoBase out"=w425, "channels"=w430, "Duration"=w427, "id"=w423, "prova.slug"=w422, "Continous?"=w421, "ByteGSAPIBase in"=w420) -> (w429:T6)
            n169 = call <vilib>:"Enqueue.vi"("error in (no error)"=w433, "data"=w429, "message"="Init", "queue in"=w424) -> ("error out"=w432:errorcluster)  [unwired: 5 in, 2 out]
          }
        }
      }
      frame "Stop Sequence" {
        n170 = Unbundle By Name(w435) -> ("queue out"=w436:refnum<queue>)
        n171 = call <vilib>:"Enqueue.vi"("High priority (F)"=TRUE, "data"=w438, "message"="Kill", "queue in"=w436) -> ("error out"=w437:errorcluster)  [unwired: 5 in, 2 out]
      }
      frame "Send Acquisition" {
        n172 = Unbundle By Name(w442) -> ("ByteGSAPIBase in"=w443:refnum<class "ByteGSAPIBase.lvclass">)
        n173 = Variant To Data(error in=w450, type=T2 {"tags"={"step_id"=0, "test_slug"="", "asset_slug"=""}, "acquisitions"=[]} ("Acquisitions"), Variant=w449) -> (data=w446:T2, error out=w447:errorcluster)
        n174 = disable-structure shown="Enabled" {
          disable-tunnel: w443 -> [w455 _]
          disable-tunnel: w447 -> [w454 _]
          disable-tunnel: w446 -> [w453 _]
          disable-tunnel: [w452 _] -> w440
          disable-tunnel: [w451 _] -> w445
          frame Enabled {
            n175 = call-dynamic "UploadAcquisitions.vi"("error in (no error)"=w454, "Acquisitions"=w453, "ByteGSAPIBase in"=w455) -> ("error out"=w451:errorcluster, "ByteGSAPIBase out"=w452:refnum<class "ByteGSAPIBase.lvclass">)  [unwired: 7 in]
          }
          frame Disabled {
          }
        }
        n176 = call <vilib>:"Clear Errors.vi"("error in (no error)"=w445) -> ("error out"=w444:errorcluster)  [unwired: 5 in, 1 out]
        n177 = Bundle By Name(cluster=w442, "ByteGSAPIBase in"=w440) -> (w441:T5)
      }
      frame "MultiStart" {
        n178 = Unbundle By Name(w468) -> ("ByteGSAPIBase in"=w469:refnum<class "ByteGSAPIBase.lvclass">, "Slug"=w462:string, "ChannelsRepoBase out"=w461:refnum<class "ChannelsRepoXML.lvclass">, "queue out"=w459:refnum<queue>)
        n179 = call "GetChannelList.vi"("error in (no error)"=w470, "ByteGSAPIBase in"=w469) -> ("error out"=w460:errorcluster, "Channels"=w465:cluster{"fields":string[]}, "ByteGSAPIBase out"=w463:refnum<class "ByteGSAPIBase.lvclass">)  [unwired: 7 in]
        n180 = Unbundle By Name(w465) -> ("fields"=w464:string[])
        n181 = Bundle By Name(cluster=T10 {"ChannelsRepoBase out"=refnum, "channels"=[], "asset_slug"="", "ByteGSAPIBase in"=refnum} ("output cluster"), "ChannelsRepoBase out"=w461, "channels"=w464, "asset_slug"=w462, "ByteGSAPIBase in"=w463) -> (w458:T10)
        n182 = call <vilib>:"Enqueue.vi"("error in (no error)"=w460, "data"=w458, "message"="Init", "queue in"=w459) -> ("error out"=w457:errorcluster)  [unwired: 5 in, 2 out]
        n183 = Bundle By Name(cluster=w468, "ByteGSAPIBase in"=w463) -> (w467:T5)
      }
      frame "KillMulti" {
        n184 = Unbundle By Name(w473) -> ("queue out"=w472:refnum<queue>)
        n185 = call <vilib>:"Enqueue.vi"("High priority (F)"=TRUE, "error in (no error)"=w475, "message"="Kill", "queue in"=w472) -> ("error out"=w474:errorcluster)  [unwired: 5 in, 2 out]
      }
    }
  }
